vi "RemoteVI Test Bytes To Hex.vi"(0 "bytes":string) -> (4 "hex":string)   [LabVIEW 2020]
doc: "Test support: renders bytes as lowercase hex, two digits per byte, the notation of tests/vectors. Pure."
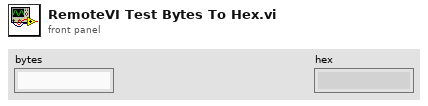
[diagram p1: front panel]
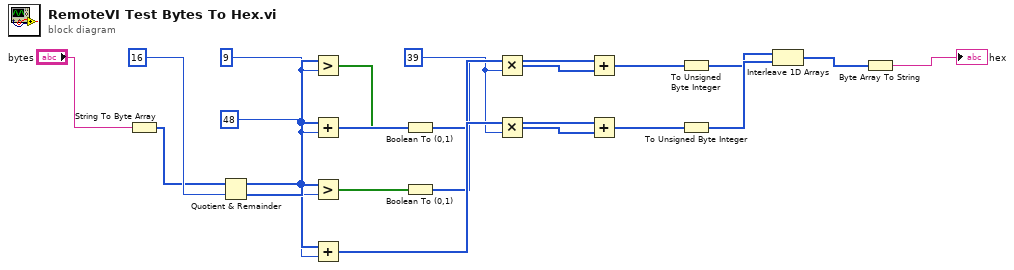
[diagram p0: block diagram]
diagram:
  w6 = u8 39
  w5 = u8 48
  w4 = u8 9
  n1 = String To Byte Array(string="bytes") -> (unsigned byte array=w2:u8[])
  n2 = Quotient & Remainder(x=w2, y=u8 16) -> (x-y*floor(x/y)=w7:u8[], floor(x/y)=w8:u8[])
  n3 = Greater?(x=w8, y=w4) -> (0:w9:bool[])
  n4 = Add(x=w8, y=w5) -> (x+y=w12:u8[])
  n5 = Greater?(x=w7, y=w4) -> (0:w15:bool[])
  n6 = Add(x=w7, y=w5) -> (x+y=w18:u8[])
  n7 = Boolean To (0,1)(Boolean=w9) -> (0, 1=w10:i16[])
  n8 = Boolean To (0,1)(Boolean=w15) -> (0, 1=w16:i16[])
  n9 = Multiply(x=w10, y=w6) -> (x*y=w11:i16[])
  n10 = Multiply(x=w16, y=w6) -> (x*y=w17:i16[])
  n11 = Add(x=w12, y=w11) -> (x+y=w13:i16[])
  n12 = Add(x=w18, y=w17) -> (x+y=w19:i16[])
  n13 = To Unsigned Byte Integer(number=w13) -> (unsigned 8bit integer=w14:u8[])
  n14 = To Unsigned Byte Integer(number=w19) -> (unsigned 8bit integer=w20:u8[])
  n15 = Interleave 1D Arrays(w14, w20) -> (w21:u8[])
  n16 = Byte Array To String(unsigned byte array=w21) -> (string=→"hex":string)
